vi "usbpt104ChannelSetting.vi"(8 "error in (no error)":errorcluster, 10 "Channel Settings":T1={"CH1 # Wires"=4, "CH1 Measurement Type"=1, "CH2 # Wires"=2, "CH2 Measurement Type"=0, "CH3 # Wires"=2, "CH3 Measurement Type"=0, "CH4 # Wires"=2, "CH4 Measurement Type"=0} {"CH4 Measurement Type" items=["OFF", "PT100", "PT1000", "Resistance to 375 Ohms", "Resistance to 10 kOhms", "Differential to 115 mV", "Differential to 2500 mV", "Single-ended to 115 mV", "Single-ended to 2500 mV"]; "CH4 # Wires" items=["2"=2, "3"=3, "4"=4]; "CH3 Measurement Type" items=["OFF", "PT100", "PT1000", "Resistance to 375 Ohms", "Resistance to 10 kOhms", "Differential to 115 mV", "Differential to 2500 mV", "Single-ended to 115 mV", "Single-ended to 2500 mV"]; "CH3 # Wires" items=["2"=2, "3"=3, "4"=4]; "CH2 Measurement Type" items=["OFF", "PT100", "PT1000", "Resistance to 375 Ohms", "Resistance to 10 kOhms", "Differential to 115 mV", "Differential to 2500 mV", "Single-ended to 115 mV", "Single-ended to 2500 mV"]; "CH2 # Wires" items=["2"=2, "3"=3, "4"=4]; "CH1 Measurement Type" items=["OFF", "PT100", "PT1000", "Resistance to 375 Ohms", "Resistance to 10 kOhms", "Differential to 115 mV", "Differential to 2500 mV", "Single-ended to 115 mV", "Single-ended to 2500 mV"]; "CH1 # Wires" items=["2"=2, "3"=3, "4"=4]}, 11 "Handle In":i16) -> (0 "error out":errorcluster, 2 "Channel Enable Array":u8[](array[numeric]), 3 "Handle out":i16)   [LabVIEW 2010]
uses:
  UsbPT104.dll
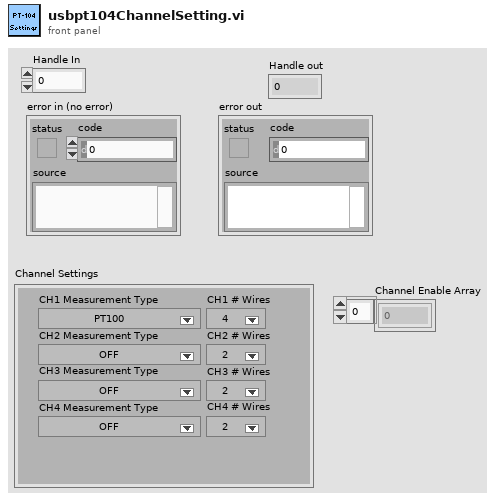
[diagram p1: front panel]
types:
  T1 = cluster{"CH1 # Wires":i16, "CH1 Measurement Type":i32, "CH2 # Wires":i16, "CH2 Measurement Type":i32, "CH3 # Wires":i16, "CH3 Measurement Type":i32, "CH4 # Wires":i16, "CH4 Measurement Type":i32}
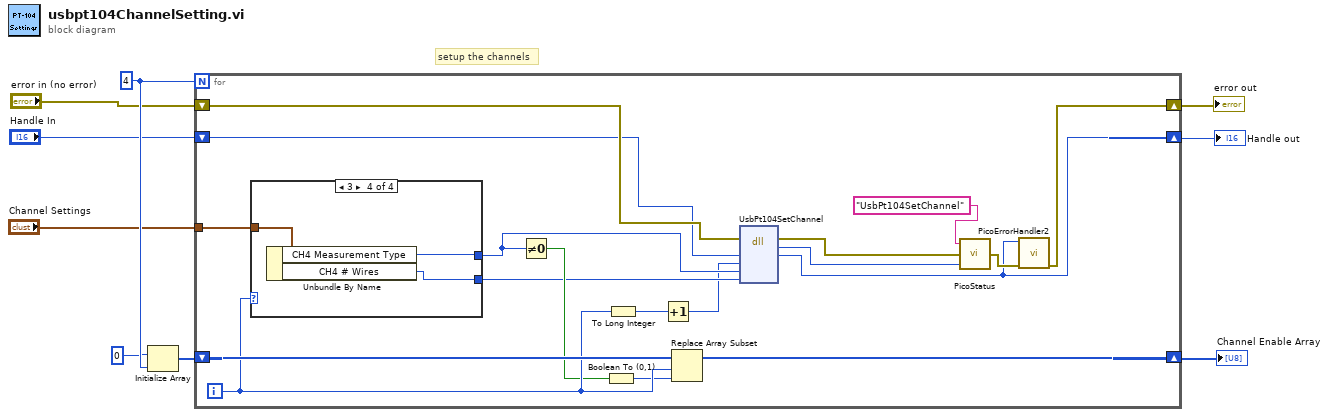
[diagram p0: block diagram]
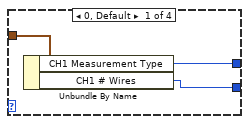
[diagram p2: hidden frame]
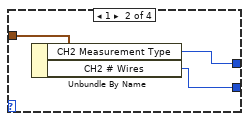
[diagram p3: hidden frame]
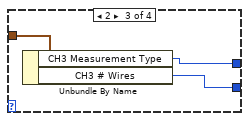
[diagram p4: hidden frame]
diagram:
  w8 = 4
  # "setup the channels"
  n1 = Initialize Array(u8 0 ("element"), w8) -> (w6:u8[])
  n2 = for {
    N: w8 -> [_]
    shift-right: [w27] -> w9
    shift-left: w6 -> [w26]
    shift-right: [w12] -> w5
    shift-left: "Handle In" -> [w22]
    shift-right: [w13] -> w1
    shift-left: "error in (no error)" -> [w23]
    tunnel: "Channel Settings" -> [w21]
    i -> [w25]
    n3 = case shown="3" w25 {
      tunnel: w21 -> [w30 w33 w36 w39]
      tunnel: [w29 w31 w35 w37] -> w17
      tunnel: [w28 w32 w34 w38] -> w16
      frame 0, Default {
        n4 = Unbundle By Name(w30) -> ("CH1 Measurement Type"=w29:i32, "CH1 # Wires"=w28:i16)
      }
      frame 1 {
        n5 = Unbundle By Name(w33) -> ("CH2 Measurement Type"=w31:i32, "CH2 # Wires"=w32:i16)
      }
      frame 2 {
        n6 = Unbundle By Name(w36) -> ("CH3 Measurement Type"=w35:i32, "CH3 # Wires"=w34:i16)
      }
      frame 3 {
        n7 = Unbundle By Name(w39) -> ("CH4 Measurement Type"=w37:i32, "CH4 # Wires"=w38:i16)
      }
    }
    n8 = Not Equal To 0?(x=w17) -> (x != 0?=w18:bool)
    n9 = Boolean To (0,1)(Boolean=w18) -> (0, 1=w24:i16)
    n10 = To Long Integer(number=w25) -> (32bit integer=w11:i32)
    n11 = Increment(x=w11) -> (x+1=w10:i32)
    n12 = Replace Array Subset(array=w26, new element=w24, index=w25) -> (w27:u8[])
    n13 = dll-call lib="UsbPT104.dll" fn="UsbPt104SetChannel"(error in=w23, "handle"=w22, "channel"=w10, "type"=w17, "noOfWires"=w16) -> (error out=w15:errorcluster, "PICO_STATUS"=w14:u32, "handle"=w12:i16)  [unwired: 5 in, 1 out]
    n14 = call "PicoStatus.vi"("PICO STATUS"=w14, "error in"=w15, "source"="UsbPt104SetChannel") -> ("error out"=w20:errorcluster)
    n15 = call "PicoErrorHandler2.vi"("error in (no error)"=w20, "handle In"=w12) -> ("error out"=w13:errorcluster)  [unwired: 9 in]
  }
  "Channel Enable Array" <- w9
  "Handle out" <- w5
  "error out" <- w1
